vi "Pre Launch Init.vi"(11 "ZM-HWM-hardware_manager in":refnum<class "ZM-HWM-hardware_manager.lvclass">) -> (0 "error out":errorcluster, 3 "ZM-HWM-hardware_manager out":refnum<class "ZM-HWM-hardware_manager.lvclass">)   [LabVIEW 2020, in "ZM-HWM-hardware_manager.lvlib" / "ZM-HWM-hardware_manager.lvclass"]
doc: "Pre Launch Init override of the hardware manager: Call Parent, then ZM-HWM-createResources creates the stop user event. If that fails, what was created is destroyed and the error fails the launch (Stop Core does not run)."
uses:
  ZM-HWM-hardware_manager.lvclass
  <vilib>/ActorFramework/Actor/Actor.lvclass
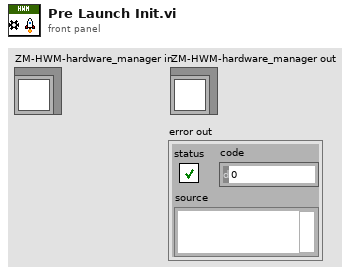
[diagram p1: front panel]
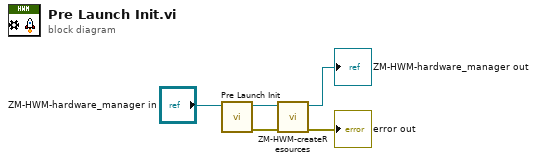
[diagram p0: block diagram]
diagram:
  n1 = call-parent "Pre Launch Init.vi"("Actor in"="ZM-HWM-hardware_manager in") -> ("error out"=w1:errorcluster, "Actor out"=w3:refnum<class "ZM-HWM-hardware_manager.lvclass">)  [unwired: 9 in]
  n2 = call "ZM-HWM-createResources.vi"("error in (no error)"=w1, "ZM-HWM-hardware_manager in"=w3) -> ("error out"=→"error out":errorcluster, "ZM-HWM-hardware_manager out"=→"ZM-HWM-hardware_manager out":refnum<class "ZM-HWM-hardware_manager.lvclass">)  [unwired: 8 in]
